vi "GCSTranslator DLL Functions.vi"(0 "System no.":i32=1 min=1 step=1, 1 "Function":T1(ring), 3 "DLL Path (Required for Application, \nmust be set once for the application)":path, 4 "String input":string, 5 "error in":errorcluster, 6 "String buffer":string, 7 "Numerical input":i32, 8 "String input 2":string) -> (14 "DLL I32 Return value":i32, 15 "Boolean output":bool, 16 "String output":string, 17 "Numerical output":i32, 19 "error out":errorcluster)   [LabVIEW 2020]
doc: "This VI calls a given function from GCSTranslator.dll. GCSTranslator.dll must be installed. To call a system-specific function, the system-specific GCS DLL must be installed also. \n\nWarning: For XXX_GcsGetANswer , String buffer must be large enough, otherwise the application may crash. Call XXX_GcsGetANswerSize first to determine necessary string length."
uses:
  Global1.vi
  Global DaisyChain.vi
panel:
  # "This vi calls a given function from GCSTranslator.dll. GCSTranslator.dll must be installed. \nThe system specific GCS DLL must be installed also.\nWARNING: For \"XXXX_GcsGetAnswer\" \"String buffer\" must be large enough, otherwise the \napplication may crash. Call \"XXXX_GcsGetAnswerSize\" first to determine necessary string length."
  # "General inputs:"
  # "Function specific inputs:"
  # "Error handling:"
  # "DLL outputs:"
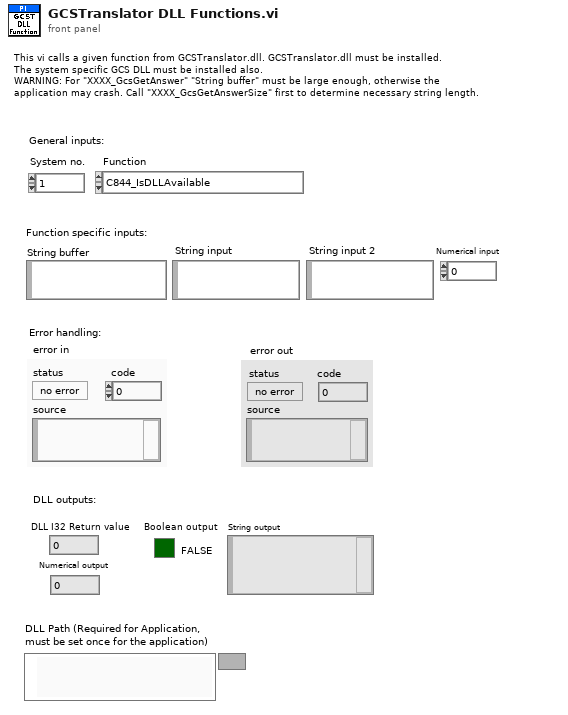
[diagram p1: front panel]
types:
  T1 = enum16{"C844_IsDLLAvailable", "C844_ConnectRS232", "C844_ConnectNIgpib", "C844_IsConnected", "C844_CloseConnection", "C844_GcsCommandset", "C844_GetError", "C844_GcsGetAnswerSize", "C844_GcsGetAnswer", "C843_IsDLLAvailable", "C843_Connect", "C843_IsConnected", "C843_CloseConnection", "C843_GcsCommandset", "C843_GetError", "C843_GcsGetAnswerSize", "C843_GcsGetAnswer", "E710_IsDLLAvailable", "E710_ConnectRS232", "E710_ConnectNIgpib", "E710_IsConnected", "E710_CloseConnection", "E710_GcsCommandset", "E710_GetError", "E710_GcsGetAnswerSize", "E710_GcsGetAnswer", "C843_PM_IsDLLAvailable", "C843_PM_Connect", "C843_PM_IsConnected", "C843_PM_CloseConnection", "C843_PM_GcsCommandset", "C843_PM_GetError", "C843_PM_GcsGetAnswerSize", "C843_PM_GcsGetAnswer", "C843_PM_GetCurrentBoardID", "C843_GetCurrentBoardID", "C865_IsDLLAvailable", "C865_ConnectRS232", "C865_IsConnected", "C865_CloseConnection", "C865_GcsCommandset", "C865_GetError", "C865_GcsGetAnswerSize", "C865_GcsGetAnswer", "C865_GetCurrentInterfaceID", "E761_ConnectPciBoard", "DefineSystem", "CloseConnection", "IsConnected", "ConnectRS232", "ConnectNIgpib", "ConnectPciBoard", "ConnectTCPIP", "GetError", "GcsCommandset", "GCSGetAnswerSize", "GcsGetAnswer", "CloseDaisyChain", "OpenRS232DaisyChain", "ConnectDaisyChainDevice", "ConnectUSB", "ListUSB", "OpenUSBDaisyChain", "OpenTCPIPDaisyChain"}
  T2 = typedef "Available interfaces.ctl" = u16
  T3 = cluster{"RS232 Portnumber":i32, "Timeout":i32, "RS232 Baud rate":u32, "Interface":T2, "GPIB Bus":i32, "GPIB Address":i32, "GPIB Mode":i32}[]
  T4 = cluster{"RS232 Portnumber":i32, "Timeout":i32, "RS232 Baud rate":u32, "Interface":T2, "GPIB Bus":i32, "GPIB Address":i32, "GPIB Mode":i32}
  T5 = typedef "Available DLLs.ctl" = u16
  T6 = typedef "Available DLL interfaces.ctl" = u16
  T7 = cluster{"DLL for Device":T5, "DLL Interface":T6, "Parameter":string}[]
  T8 = cluster{"DLL for Device":T5, "DLL Interface":T6, "Parameter":string}
  T9 = cluster{"No. of devices":i32, "Port ID":i32, "Devices":string[], "Description":string}[]
  T10 = cluster{"No. of devices":i32, "Port ID":i32, "Devices":string[], "Description":string}
  T11 = cluster{"Host address/name":string, "Port":i32, "Board":i32}[]
  T12 = cluster{"Host address/name":string, "Port":i32, "Board":i32}
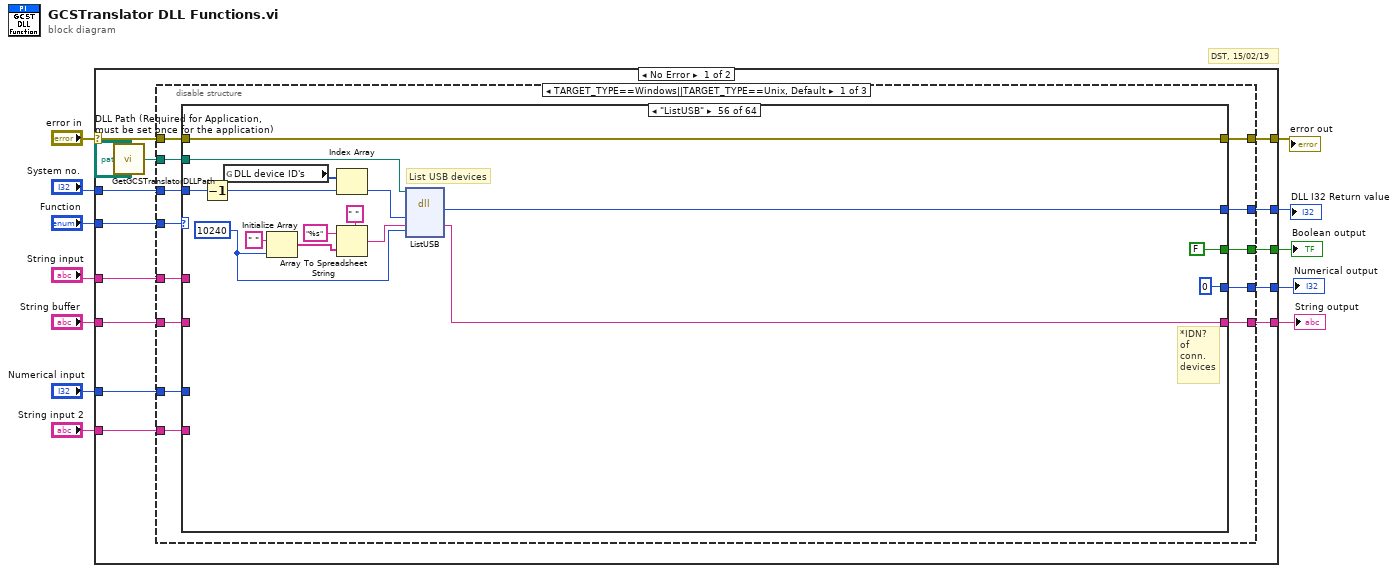
[diagram p0: block diagram]
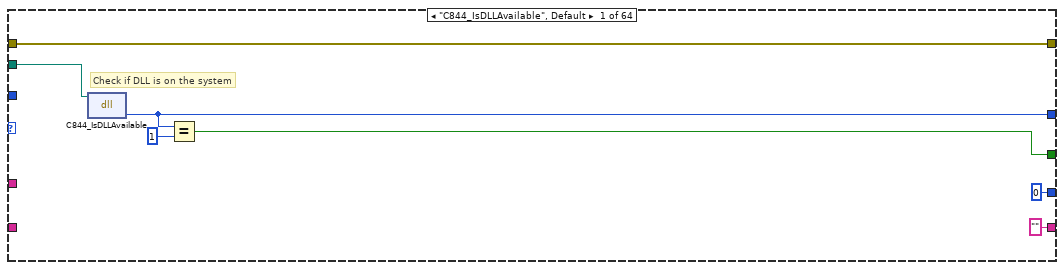
[diagram p2: hidden frame]
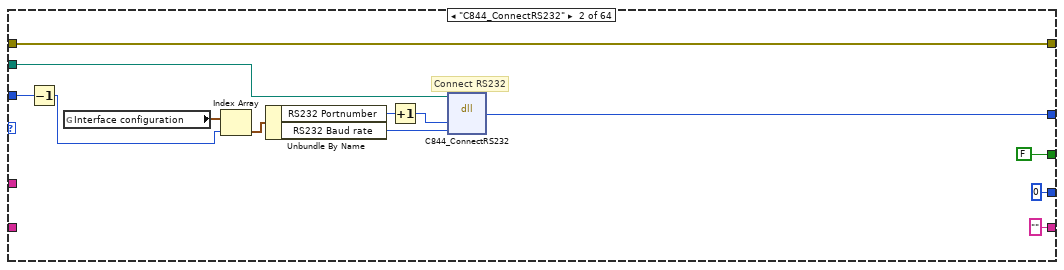
[diagram p3: hidden frame]
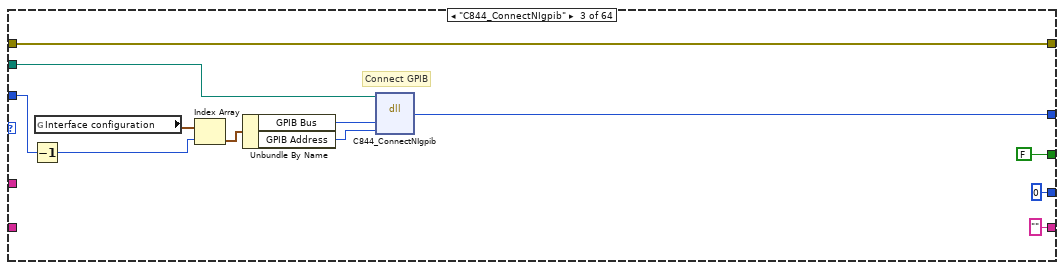
[diagram p4: hidden frame]
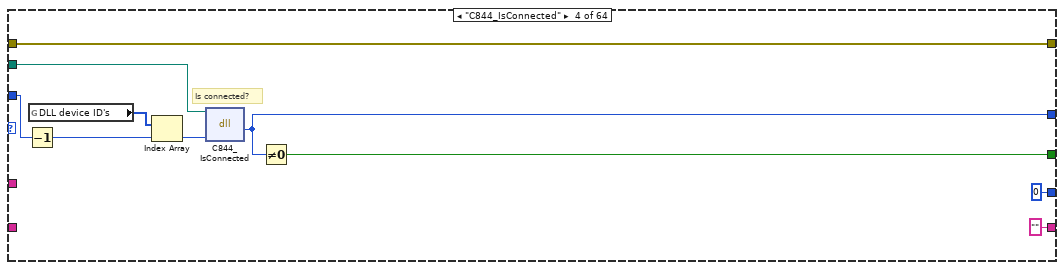
[diagram p5: hidden frame]
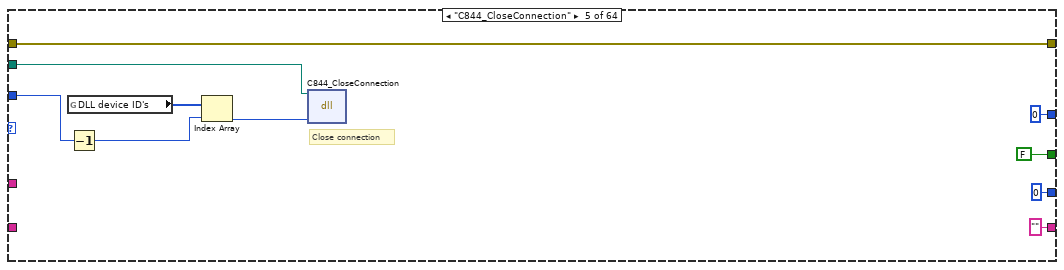
[diagram p6: hidden frame]
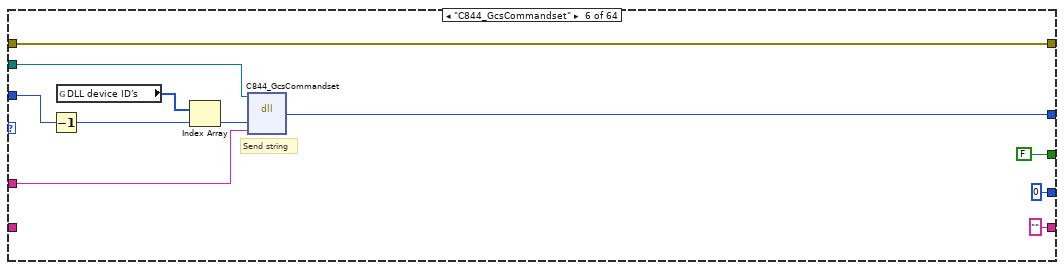
[diagram p7: hidden frame]
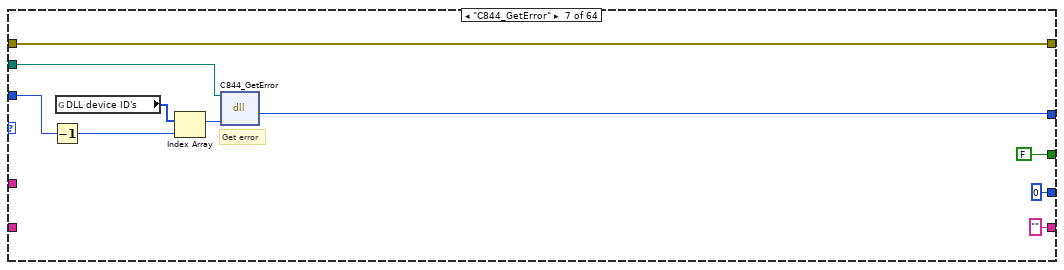
[diagram p8: hidden frame]
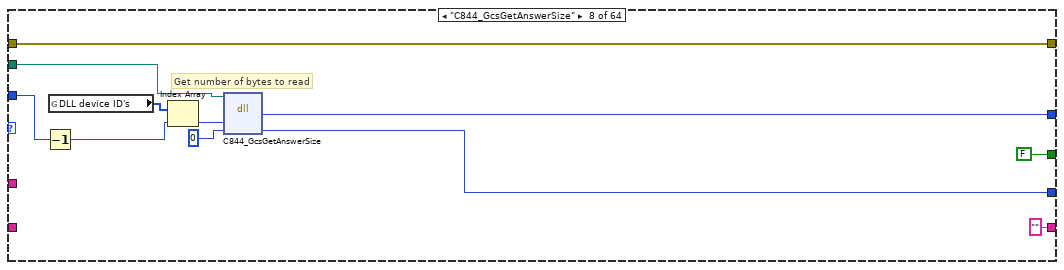
[diagram p9: hidden frame]
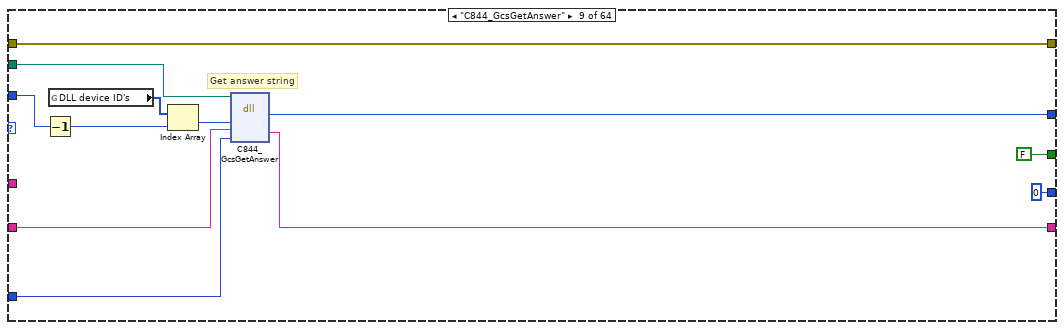
[diagram p10: hidden frame]
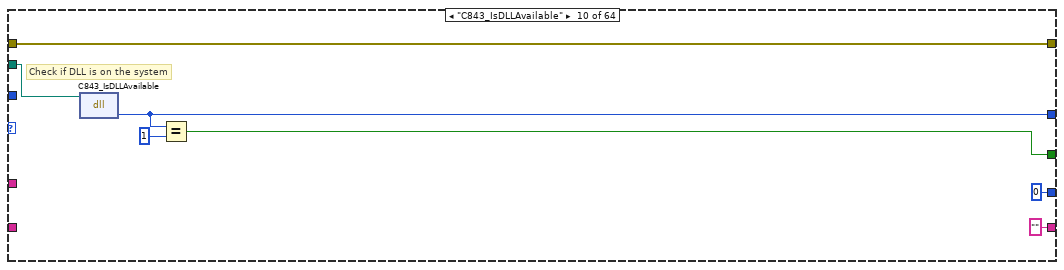
[diagram p11: hidden frame]
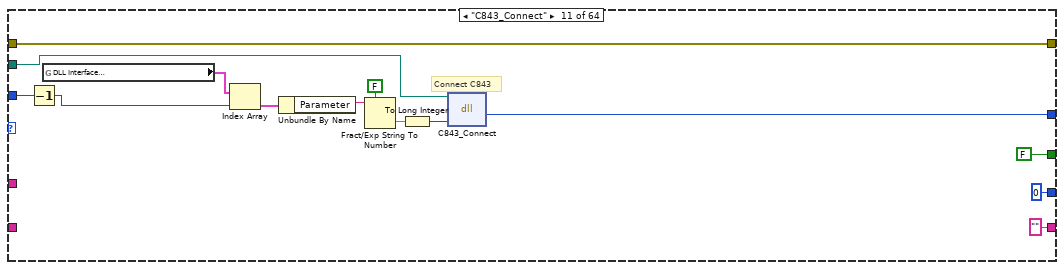
[diagram p12: hidden frame]
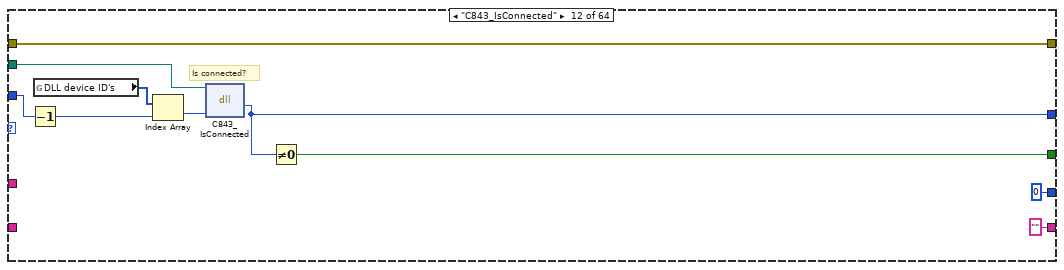
[diagram p13: hidden frame]
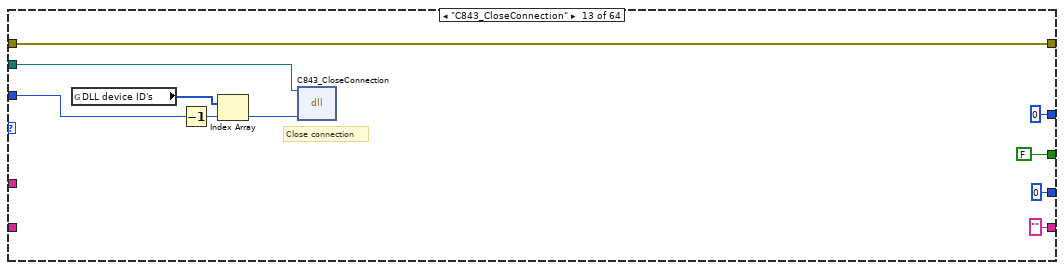
[diagram p14: hidden frame]
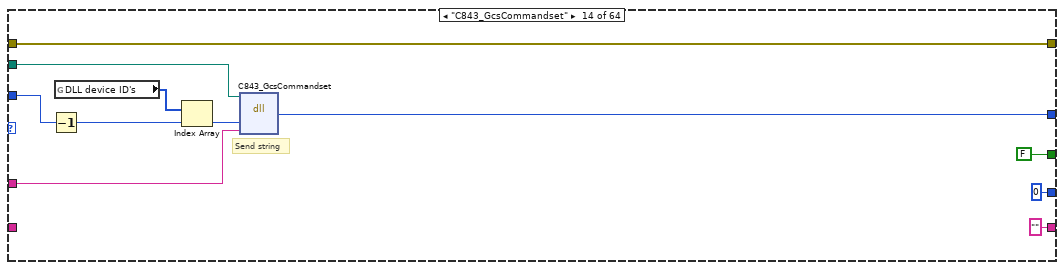
[diagram p15: hidden frame]
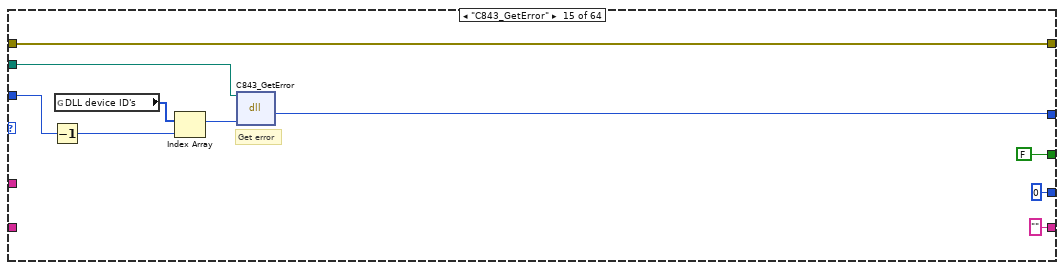
[diagram p16: hidden frame]
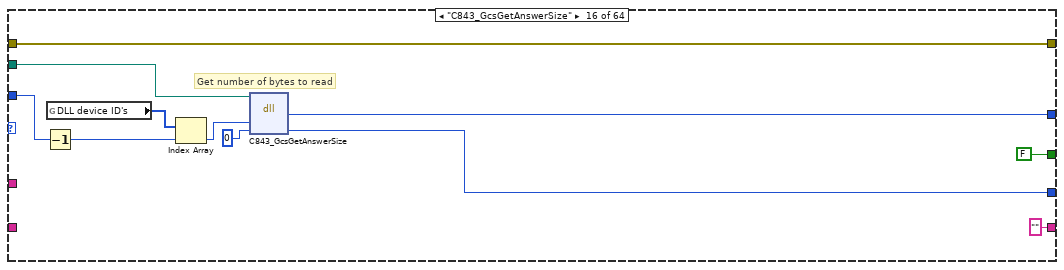
[diagram p17: hidden frame]
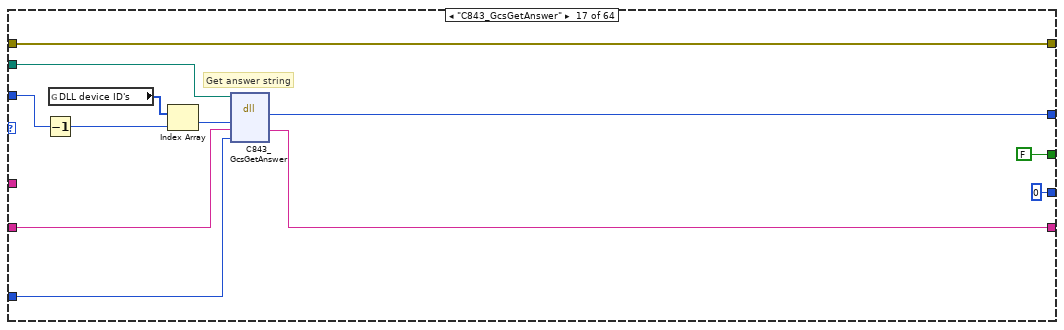
[diagram p18: hidden frame]
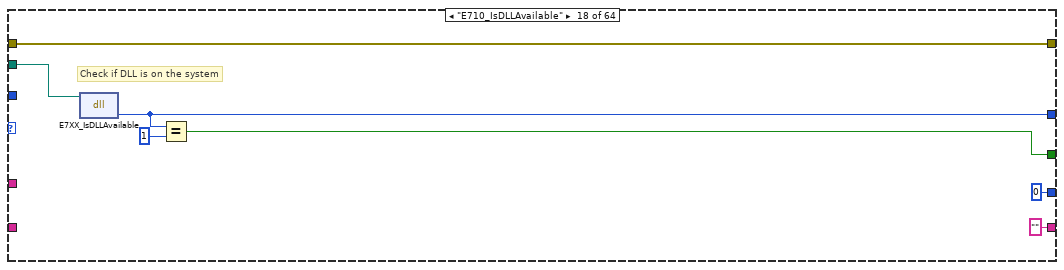
[diagram p19: hidden frame]
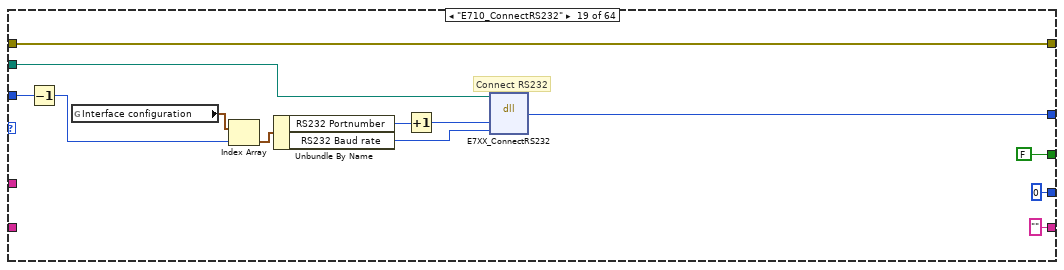
[diagram p20: hidden frame]
diagram:
  # "DST, 15/02/19"
  n1 = case shown="No Error" "error in" {
    selector: "error in" -> [w17 w892]
    tunnel: [w26 w892] -> w12
    tunnel: [w25 0] -> w11
    tunnel: [w24 FALSE] -> w10
    tunnel: "String input" -> [w23 _]
    tunnel: [w22 0 ("iAnswerSize")] -> w8
    tunnel: "String buffer" -> [w21 _]
    tunnel: [w20 "" ("szAnswer")] -> w6
    tunnel: "Numerical input" -> [w19 _]
    tunnel: "String input 2" -> [w18 _]
    tunnel: "System no." -> [w16 _]
    tunnel: "Function" -> [w15 _]
    frame No Error {
      n2 = call "GetGCSTranslatorDLLPath.vi"("DLL Path (Required for Application, \nmust be set once for the application)"="DLL Path (Required for Application, \nmust be set once for the application)") -> ("DLL path"=w14:path)
      n3 = disable-structure shown="TARGET_TYPE==Windows||TARGET_TYPE==Unix, Default" {
        disable-tunnel: w15 -> [w39 _ _]
        disable-tunnel: w17 -> [w38 w890 w891]
        disable-tunnel: [w37 w890 w891] -> w26
        disable-tunnel: [w36 _ _] -> w25
        disable-tunnel: w16 -> [w35 _ _]
        disable-tunnel: [w34 _ _] -> w24
        disable-tunnel: w23 -> [w33 _ _]
        disable-tunnel: [w32 _ _] -> w22
        disable-tunnel: w21 -> [w31 _ _]
        disable-tunnel: [w30 _ _] -> w20
        disable-tunnel: w19 -> [w29 _ _]
        disable-tunnel: w18 -> [w28 _ _]
        disable-tunnel: w14 -> [w27 _ _]
        frame condition #0 (active) {
          n4 = case shown="\"ListUSB\"" w39 {
            tunnel: w35 -> [_ w53 w66 w76 w86 w97 w107 w117 w130 _ w153 w161 w171 w182 w192 w202 w215 _ w234 w247 w257 w267 w278 w288 w298 w311 _ w335 w342 w352 w363 w373 w383 w396 w412 w426 _ w444 w454 w464 w475 w485 w495 w508 w524 _ w540 w548 w583 w600 w622 w651 w701 w734 w763 w779 w791 w807 w821 w835 w846 w861 w871 w884]
            tunnel: w38 -> [w46 w51 w64 w79 w91 w102 w112 w123 w135 w142 w151 w164 w176 w187 w197 w208 w220 w227 w232 w245 w260 w272 w283 w293 w304 w316 w323 w333 w345 w357 w368 w378 w389 w401 w410 w424 w436 w442 w457 w469 w480 w490 w501 w513 w522 w532 w545 w561 w586 w598 w608 w642 w700 w733 w762 w778 w789 w805 w819 w834 w841 w866 w877 w889]
            tunnel: [w46 w51 w64 w79 w91 w102 w112 w123 w135 w142 w151 w164 w176 w187 w197 w208 w220 w227 w232 w245 w260 w272 w283 w293 w304 w316 w323 w333 w345 w357 w368 w378 w389 w401 w410 w424 w436 w442 w457 w469 w480 w490 w501 w513 w522 w532 w545 w561 w586 w598 w607 w641 w700 w733 w762 w778 w789 w805 w819 w834 w840 w866 w877 w889] -> w37
            tunnel: [w45 w52 w65 w78 0 w101 w111 w121 w134 w141 w152 w163 0 w186 w196 w206 w219 w226 w233 w246 w259 0 w282 w292 w302 w315 w322 w334 w344 0 w367 w377 w387 w400 w411 w425 w435 w443 w456 0 w479 w489 w499 w512 w523 w533 0 0 w585 w599 w621 w650 w677 w716 w751 w769 w790 w806 w820 w828 w839 w865 w875 w888] -> w36
            tunnel: [w43 FALSE FALSE w75 FALSE FALSE FALSE FALSE FALSE w139 FALSE w160 FALSE FALSE FALSE FALSE FALSE w224 FALSE FALSE w256 FALSE FALSE FALSE FALSE FALSE w320 FALSE w341 FALSE FALSE FALSE FALSE FALSE FALSE FALSE w433 FALSE w453 FALSE FALSE FALSE FALSE FALSE FALSE FALSE FALSE FALSE w582 FALSE FALSE FALSE FALSE FALSE FALSE FALSE FALSE FALSE FALSE FALSE FALSE FALSE FALSE FALSE] -> w34
            tunnel: w33 -> [_ _ _ _ _ w95 _ _ _ _ _ _ _ w180 _ _ _ _ _ _ _ _ w276 _ _ _ _ _ _ _ w361 _ _ _ _ _ _ _ _ _ w473 _ _ _ _ w535 _ _ _ _ _ _ _ _ _ _ _ _ _ _ _ w859 _ _]
            tunnel: [0 ("iAnswerSize") 0 ("iAnswerSize") 0 ("iAnswerSize") 0 ("iAnswerSize") 0 ("iAnswerSize") 0 ("iAnswerSize") 0 ("iAnswerSize") w115 0 ("iAnswerSize") 0 ("iAnswerSize") 0 ("iAnswerSize") 0 ("iAnswerSize") 0 ("iAnswerSize") 0 ("iAnswerSize") 0 ("iAnswerSize") w200 0 ("iAnswerSize") 0 ("iAnswerSize") 0 ("iAnswerSize") 0 ("iAnswerSize") 0 ("iAnswerSize") 0 ("iAnswerSize") 0 ("iAnswerSize") 0 ("iAnswerSize") w296 0 ("iAnswerSize") 0 ("iAnswerSize") 0 ("iAnswerSize") 0 ("iAnswerSize") 0 ("iAnswerSize") 0 ("iAnswerSize") 0 ("iAnswerSize") w381 0 ("iAnswerSize") 0 ("iAnswerSize") 0 ("iAnswerSize") 0 ("iAnswerSize") 0 ("iAnswerSize") 0 ("iAnswerSize") 0 ("iAnswerSize") 0 ("iAnswerSize") 0 ("iAnswerSize") w493 0 ("iAnswerSize") 0 ("iAnswerSize") 0 ("iAnswerSize") 0 ("iAnswerSize") 0 ("iAnswerSize") 0 ("iAnswerSize") 0 ("iAnswerSize") 0 ("iAnswerSize") 0 ("iAnswerSize") w676 w715 w748 0 ("iAnswerSize") 0 ("iAnswerSize") 0 ("iAnswerSize") 0 ("iAnswerSize") 0 ("iAnswerSize") 0 ("iAnswerSize") 0 ("iAnswerSize") w869 0 ("iAnswerSize")] -> w32
            tunnel: w31 -> [_ _ _ _ _ _ _ _ w128 _ _ _ _ _ _ _ w213 _ _ _ _ _ _ _ _ w309 _ _ _ _ _ _ _ w394 _ _ _ _ _ _ _ _ _ w506 _ _ _ _ _ _ _ _ _ _ _ _ _ _ _ _ _ _ _ w882]
            tunnel: ["" ("szAnswer") "" ("szAnswer") "" ("szAnswer") "" ("szAnswer") "" ("szAnswer") "" ("szAnswer") "" ("szAnswer") "" ("szAnswer") w127 "" ("szAnswer") "" ("szAnswer") "" ("szAnswer") "" ("szAnswer") "" ("szAnswer") "" ("szAnswer") "" ("szAnswer") w212 "" ("szAnswer") "" ("szAnswer") "" ("szAnswer") "" ("szAnswer") "" ("szAnswer") "" ("szAnswer") "" ("szAnswer") "" ("szAnswer") w308 "" ("szAnswer") "" ("szAnswer") "" ("szAnswer") "" ("szAnswer") "" ("szAnswer") "" ("szAnswer") "" ("szAnswer") w393 "" ("szAnswer") "" ("szAnswer") "" ("szAnswer") "" ("szAnswer") "" ("szAnswer") "" ("szAnswer") "" ("szAnswer") "" ("szAnswer") "" ("szAnswer") w505 "" ("szAnswer") "" ("szAnswer") "" ("szAnswer") "" ("szAnswer") "" ("szAnswer") "" ("szAnswer") "" ("szAnswer") "" ("szAnswer") w675 w714 w746 w767 "" ("szAnswer") "" ("szAnswer") "" ("szAnswer") "" ("szAnswer") "" ("szAnswer") "" ("szAnswer") "" ("szAnswer") w881] -> w30
            tunnel: w29 -> [_ _ _ _ _ _ _ _ w125 _ _ _ _ _ _ _ w210 _ _ _ _ _ _ _ _ w306 _ _ _ _ _ _ _ w391 _ _ _ _ _ _ _ _ _ w503 _ _ _ _ _ _ _ _ _ _ _ _ _ _ _ _ _ _ _ w879]
            tunnel: w28 -> [_ _ _ _ _ _ _ _ _ _ _ _ _ _ _ _ _ _ _ _ _ _ _ _ _ _ _ _ _ _ _ _ _ _ _ _ _ _ _ _ _ _ _ _ _ w534 _ _ _ _ _ _ _ _ _ _ _ _ _ _ _ _ _ _]
            tunnel: w27 -> [w40 w47 w60 w72 w82 w92 w103 w113 w124 w136 w143 w157 w167 w177 w188 w198 w209 w221 w228 w241 w253 w263 w273 w284 w294 w305 w317 w324 w338 w348 w358 w369 w379 w390 w402 w416 w430 w437 w450 w460 w470 w481 w491 w502 w514 w528 w536 w546 w579 w589 w604 w631 w666 w705 w737 w764 w780 w794 w810 w824 w838 w856 w867 w878]
            frame "C844_IsDLLAvailable", Default {
              # "Check if DLL is on the system"
              n5 = dll-call lib="T:/Entwicklung/HostSoftware/LabVIEW/GCSDrivers/source/GCS2LabVIEW/Low Level/GCSTranslator.dll" fn="C844_IsDLLAvailable"(path in=w40) -> ("return type"=w45:i32)  [unwired: 2 in, 2 out]
              n6 = Equal?(x=w45, y=1) -> (x = y?=w43:bool)
            }
            frame "C844_ConnectRS232" {
              # "Connect RS232"
              n7 = Decrement(x=w53) -> (x-1=w55:i32)
              n8 = global read "Global1.vi" "Interface configuration"() -> (w56:T3)
              n9 = Index Array(array=w56, index=w55) -> (element=w54:T4)
              n10 = Unbundle By Name(w54) -> ("RS232 Portnumber"=w57:i32, "RS232 Baud rate"=w59:u32)
              n11 = Increment(x=w57) -> (x+1=w58:i32)
              n12 = dll-call lib="T:/Entwicklung/HostSoftware/LabVIEW/GCSDrivers/source/GCS2LabVIEW/Low Level/GCSTranslator.dll" fn="C844_ConnectRS232"(path in=w47, "nPortNr"=w58, "nBaudRate"=w59) -> ("return type"=w52:i32)  [unwired: 4 in, 2 out]
            }
            frame "C844_ConnectNIgpib" {
              # "Connect GPIB"
              n13 = Decrement(x=w66) -> (x-1=w68:i32)
              n14 = global read "Global1.vi" "Interface configuration"() -> (w69:T3)
              n15 = Index Array(array=w69, index=w68) -> (element=w67:T4)
              n16 = Unbundle By Name(w67) -> ("GPIB Bus"=w71:i32, "GPIB Address"=w70:i32)
              n17 = dll-call lib="T:/Entwicklung/HostSoftware/LabVIEW/GCSDrivers/source/GCS2LabVIEW/Low Level/GCSTranslator.dll" fn="C844_ConnectNIgpib"(path in=w60, "nBoard"=w71, "nDevAddr"=w70) -> ("return type"=w65:i32)  [unwired: 4 in, 2 out]
            }
            frame "C844_IsConnected" {
              # "Is connected?"
              n18 = Decrement(x=w76) -> (x-1=w80:i32)
              n19 = global read "Global1.vi" "DLL device ID's"() -> (w77:i32[])
              n20 = Index Array(array=w77, index=w80) -> (element=w81:i32)
              n21 = dll-call lib="T:/Entwicklung/HostSoftware/LabVIEW/GCSDrivers/source/GCS2LabVIEW/Low Level/GCSTranslator.dll" fn="C844_IsConnected"(path in=w72, "ID"=w81) -> ("return type"=w78:i32)  [unwired: 3 in, 2 out]
              n22 = Not Equal To 0?(x=w78) -> (x != 0?=w75:bool)
            }
            frame "C844_CloseConnection" {
              # "Close connection"
              n23 = global read "Global1.vi" "DLL device ID's"() -> (w88:i32[])
              n24 = Decrement(x=w86) -> (x-1=w89:i32)
              n25 = Index Array(array=w88, index=w89) -> (element=w87:i32)
              n26 = dll-call lib="T:/Entwicklung/HostSoftware/LabVIEW/GCSDrivers/source/GCS2LabVIEW/Low Level/GCSTranslator.dll" fn="C844_CloseConnection"(path in=w82, "ID"=w87) -> ()  [unwired: 3 in, 3 out]
            }
            frame "C844_GcsCommandset" {
              # "Send string"
              n27 = Decrement(x=w97) -> (x-1=w100:i32)
              n28 = global read "Global1.vi" "DLL device ID's"() -> (w99:i32[])
              n29 = Index Array(array=w99, index=w100) -> (element=w98:i32)
              n30 = dll-call lib="T:/Entwicklung/HostSoftware/LabVIEW/GCSDrivers/source/GCS2LabVIEW/Low Level/GCSTranslator.dll" fn="C844_GcsCommandset"(path in=w92, "ID"=w98, "szCommand"=w95) -> ("return type"=w101:i32)  [unwired: 4 in, 2 out]
            }
            frame "C844_GetError" {
              # "Get error"
              n31 = Decrement(x=w107) -> (x-1=w110:i32)
              n32 = global read "Global1.vi" "DLL device ID's"() -> (w109:i32[])
              n33 = Index Array(array=w109, index=w110) -> (element=w108:i32)
              n34 = dll-call lib="T:/Entwicklung/HostSoftware/LabVIEW/GCSDrivers/source/GCS2LabVIEW/Low Level/GCSTranslator.dll" fn="C844_GetError"(path in=w103, "ID"=w108) -> ("return type"=w111:i32)  [unwired: 3 in, 2 out]
            }
            frame "C844_GcsGetAnswerSize" {
              # "Get number of bytes to read"
              n35 = Decrement(x=w117) -> (x-1=w120:i32)
              n36 = global read "Global1.vi" "DLL device ID's"() -> (w119:i32[])
              n37 = Index Array(array=w119, index=w120) -> (element=w118:i32)
              n38 = dll-call lib="T:/Entwicklung/HostSoftware/LabVIEW/GCSDrivers/source/GCS2LabVIEW/Low Level/GCSTranslator.dll" fn="C844_GcsGetAnswerSize"(path in=w113, "ID"=w118, "iAnswerSize"=0) -> ("return type"=w121:i32, "iAnswerSize"=w115:i32)  [unwired: 3 in, 2 out]
            }
            frame "C844_GcsGetAnswer" {
              # "Get answer string"
              n39 = Decrement(x=w130) -> (x-1=w133:i32)
              n40 = global read "Global1.vi" "DLL device ID's"() -> (w132:i32[])
              n41 = Index Array(array=w132, index=w133) -> (element=w131:i32)
              n42 = dll-call lib="T:/Entwicklung/HostSoftware/LabVIEW/GCSDrivers/source/GCS2LabVIEW/Low Level/GCSTranslator.dll" fn="C844_GcsGetAnswer"(path in=w124, "ID"=w131, "szAnswer"=w128, "iAnswerSize"=w125) -> ("return type"=w134:i32, "szAnswer"=w127:string)  [unwired: 4 in, 2 out]
            }
            frame "C843_IsDLLAvailable" {
              # "Check if DLL is on the system"
              n43 = dll-call lib="T:/Entwicklung/HostSoftware/LabVIEW/GCSDrivers/source/GCS2LabVIEW/Low Level/GCSTranslator.dll" fn="C843_IsDLLAvailable"(path in=w136) -> ("return type"=w141:i32)  [unwired: 2 in, 2 out]
              n44 = Equal?(x=w141, y=1) -> (x = y?=w139:bool)
            }
            frame "C843_Connect" {
              # "Connect C843"
              n45 = Decrement(x=w153) -> (x-1=w155:i32)
              n46 = global read "Global1.vi" "DLL Interface\nConfiguration"() -> (w156:T7)
              n47 = Index Array(array=w156, index=w155) -> (element=w154:T8)
              n48 = Unbundle By Name(w154) -> ("Parameter"=w147:string)
              n49 = Fract/Exp String To Number(use system decimal point (T)=FALSE, string=w147) -> (number=w148:dbl)  [unwired: 3 out]
              n50 = To Long Integer(number=w148) -> (32bit integer=w146:i32)
              n51 = dll-call lib="T:/Entwicklung/HostSoftware/LabVIEW/GCSDrivers/source/GCS2LabVIEW/Low Level/GCSTranslator.dll" fn="C843_Connect"(path in=w143, "iBoardNumber"=w146) -> ("return type"=w152:i32)  [unwired: 3 in, 2 out]
            }
            frame "C843_IsConnected" {
              # "Is connected?"
              n52 = Decrement(x=w161) -> (x-1=w165:i32)
              n53 = global read "Global1.vi" "DLL device ID's"() -> (w162:i32[])
              n54 = Index Array(array=w162, index=w165) -> (element=w166:i32)
              n55 = dll-call lib="T:/Entwicklung/HostSoftware/LabVIEW/GCSDrivers/source/GCS2LabVIEW/Low Level/GCSTranslator.dll" fn="C843_IsConnected"(path in=w157, "ID"=w166) -> ("return type"=w163:i32)  [unwired: 3 in, 2 out]
              n56 = Not Equal To 0?(x=w163) -> (x != 0?=w160:bool)
            }
            frame "C843_CloseConnection" {
              # "Close connection"
              n57 = global read "Global1.vi" "DLL device ID's"() -> (w173:i32[])
              n58 = Decrement(x=w171) -> (x-1=w174:i32)
              n59 = Index Array(array=w173, index=w174) -> (element=w172:i32)
              n60 = dll-call lib="T:/Entwicklung/HostSoftware/LabVIEW/GCSDrivers/source/GCS2LabVIEW/Low Level/GCSTranslator.dll" fn="C843_CloseConnection"(path in=w167, "ID"=w172) -> ()  [unwired: 3 in, 3 out]
            }
            frame "C843_GcsCommandset" {
              # "Send string"
              n61 = Decrement(x=w182) -> (x-1=w185:i32)
              n62 = global read "Global1.vi" "DLL device ID's"() -> (w184:i32[])
              n63 = Index Array(array=w184, index=w185) -> (element=w183:i32)
              n64 = dll-call lib="T:/Entwicklung/HostSoftware/LabVIEW/GCSDrivers/source/GCS2LabVIEW/Low Level/GCSTranslator.dll" fn="C843_GcsCommandset"(path in=w177, "ID"=w183, "szCommand"=w180) -> ("return type"=w186:i32)  [unwired: 4 in, 2 out]
            }
            frame "C843_GetError" {
              # "Get error"
              n65 = Decrement(x=w192) -> (x-1=w195:i32)
              n66 = global read "Global1.vi" "DLL device ID's"() -> (w194:i32[])
              n67 = Index Array(array=w194, index=w195) -> (element=w193:i32)
              n68 = dll-call lib="T:/Entwicklung/HostSoftware/LabVIEW/GCSDrivers/source/GCS2LabVIEW/Low Level/GCSTranslator.dll" fn="C843_GetError"(path in=w188, "ID"=w193) -> ("return type"=w196:i32)  [unwired: 3 in, 2 out]
            }
            frame "C843_GcsGetAnswerSize" {
              # "Get number of bytes to read"
              n69 = Decrement(x=w202) -> (x-1=w205:i32)
              n70 = global read "Global1.vi" "DLL device ID's"() -> (w204:i32[])
              n71 = Index Array(array=w204, index=w205) -> (element=w203:i32)
              n72 = dll-call lib="T:/Entwicklung/HostSoftware/LabVIEW/GCSDrivers/source/GCS2LabVIEW/Low Level/GCSTranslator.dll" fn="C843_GcsGetAnswerSize"(path in=w198, "ID"=w203, "iAnswerSize"=0) -> ("return type"=w206:i32, "iAnswerSize"=w200:i32)  [unwired: 3 in, 2 out]
            }
            frame "C843_GcsGetAnswer" {
              # "Get answer string"
              n73 = Decrement(x=w215) -> (x-1=w218:i32)
              n74 = global read "Global1.vi" "DLL device ID's"() -> (w217:i32[])
              n75 = Index Array(array=w217, index=w218) -> (element=w216:i32)
              n76 = dll-call lib="T:/Entwicklung/HostSoftware/LabVIEW/GCSDrivers/source/GCS2LabVIEW/Low Level/GCSTranslator.dll" fn="C843_GcsGetAnswer"(path in=w209, "ID"=w216, "szAnswer"=w213, "iAnswerSize"=w210) -> ("return type"=w219:i32, "szAnswer"=w212:string)  [unwired: 4 in, 2 out]
            }
            frame "E710_IsDLLAvailable" {
              # "Check if DLL is on the system"
              n77 = dll-call lib="T:/Entwicklung/HostSoftware/LabVIEW/GCSDrivers/source/GCS2LabVIEW/Low Level/GCSTranslator.dll" fn="E7XX_IsDLLAvailable"(path in=w221) -> ("return type"=w226:i32)  [unwired: 2 in, 2 out]
              n78 = Equal?(x=w226, y=1) -> (x = y?=w224:bool)
            }
            frame "E710_ConnectRS232" {
              # "Connect RS232"
              n79 = Decrement(x=w234) -> (x-1=w236:i32)
              n80 = global read "Global1.vi" "Interface configuration"() -> (w237:T3)
              n81 = Index Array(array=w237, index=w236) -> (element=w235:T4)
              n82 = Unbundle By Name(w235) -> ("RS232 Portnumber"=w238:i32, "RS232 Baud rate"=w240:u32)
              n83 = Increment(x=w238) -> (x+1=w239:i32)
              n84 = dll-call lib="T:/Entwicklung/HostSoftware/LabVIEW/GCSDrivers/source/GCS2LabVIEW/Low Level/GCSTranslator.dll" fn="E7XX_ConnectRS232"(path in=w228, "nPortNr"=w239, "nBaudRate"=w240) -> ("return type"=w233:i32)  [unwired: 4 in, 2 out]
            }
            frame "E710_ConnectNIgpib" {
              # "Connect GPIB"
              n85 = Decrement(x=w247) -> (x-1=w249:i32)
              n86 = global read "Global1.vi" "Interface configuration"() -> (w250:T3)
              n87 = Index Array(array=w250, index=w249) -> (element=w248:T4)
              n88 = Unbundle By Name(w248) -> ("GPIB Bus"=w252:i32, "GPIB Address"=w251:i32)
              n89 = dll-call lib="T:/Entwicklung/HostSoftware/LabVIEW/GCSDrivers/source/GCS2LabVIEW/Low Level/GCSTranslator.dll" fn="E7XX_ConnectNIgpib"(path in=w241, "nBoard"=w252, "nDevAddr"=w251) -> ("return type"=w246:i32)  [unwired: 4 in, 2 out]
            }
            frame "E710_IsConnected" {
              # "Is connected?"
              n90 = global read "Global1.vi" "DLL device ID's"() -> (w258:i32[])
              n91 = Decrement(x=w257) -> (x-1=w261:i32)
              n92 = Index Array(array=w258, index=w261) -> (element=w262:i32)
              n93 = dll-call lib="T:/Entwicklung/HostSoftware/LabVIEW/GCSDrivers/source/GCS2LabVIEW/Low Level/GCSTranslator.dll" fn="E7XX_IsConnected"(path in=w253, "ID"=w262) -> ("return type"=w259:i32)  [unwired: 3 in, 2 out]
              n94 = Not Equal To 0?(x=w259) -> (x != 0?=w256:bool)
            }
            frame "E710_CloseConnection" {
              # "Close connection"
              n95 = global read "Global1.vi" "DLL device ID's"() -> (w269:i32[])
              n96 = Decrement(x=w267) -> (x-1=w270:i32)
              n97 = Index Array(array=w269, index=w270) -> (element=w268:i32)
              n98 = dll-call lib="T:/Entwicklung/HostSoftware/LabVIEW/GCSDrivers/source/GCS2LabVIEW/Low Level/GCSTranslator.dll" fn="E7XX_CloseConnection"(path in=w263, "ID"=w268) -> ()  [unwired: 3 in, 3 out]
            }
            frame "E710_GcsCommandset" {
              # "Send string"
              n99 = global read "Global1.vi" "DLL device ID's"() -> (w280:i32[])
              n100 = Decrement(x=w278) -> (x-1=w281:i32)
              n101 = Index Array(array=w280, index=w281) -> (element=w279:i32)
              n102 = dll-call lib="T:/Entwicklung/HostSoftware/LabVIEW/GCSDrivers/source/GCS2LabVIEW/Low Level/GCSTranslator.dll" fn="E7XX_GcsCommandset"(path in=w273, "ID"=w279, "szCommand"=w276) -> ("return type"=w282:i32)  [unwired: 4 in, 2 out]
            }
            frame "E710_GetError" {
              # "Get error"
              n103 = Decrement(x=w288) -> (x-1=w291:i32)
              n104 = global read "Global1.vi" "DLL device ID's"() -> (w290:i32[])
              n105 = Index Array(array=w290, index=w291) -> (element=w289:i32)
              n106 = dll-call lib="T:/Entwicklung/HostSoftware/LabVIEW/GCSDrivers/source/GCS2LabVIEW/Low Level/GCSTranslator.dll" fn="E7XX_GetError"(path in=w284, "ID"=w289) -> ("return type"=w292:i32)  [unwired: 3 in, 2 out]
            }
            frame "E710_GcsGetAnswerSize" {
              # "Get number of bytes to read"
              n107 = Decrement(x=w298) -> (x-1=w301:i32)
              n108 = global read "Global1.vi" "DLL device ID's"() -> (w300:i32[])
              n109 = Index Array(array=w300, index=w301) -> (element=w299:i32)
              n110 = dll-call lib="T:/Entwicklung/HostSoftware/LabVIEW/GCSDrivers/source/GCS2LabVIEW/Low Level/GCSTranslator.dll" fn="E7XX_GcsGetAnswerSize"(path in=w294, "ID"=w299, "iAnswerSize"=0) -> ("return type"=w302:i32, "iAnswerSize"=w296:i32)  [unwired: 3 in, 2 out]
            }
            frame "E710_GcsGetAnswer" {
              # "Get answer string"
              n111 = Decrement(x=w311) -> (x-1=w314:i32)
              n112 = global read "Global1.vi" "DLL device ID's"() -> (w313:i32[])
              n113 = Index Array(array=w313, index=w314) -> (element=w312:i32)
              n114 = dll-call lib="T:/Entwicklung/HostSoftware/LabVIEW/GCSDrivers/source/GCS2LabVIEW/Low Level/GCSTranslator.dll" fn="E7XX_GcsGetAnswer"(path in=w305, "ID"=w312, "szAnswer"=w309, "iAnswerSize"=w306) -> ("return type"=w315:i32, "szAnswer"=w308:string)  [unwired: 4 in, 2 out]
            }
            frame "C843_PM_IsDLLAvailable" {
              # "Check if DLL is on the system"
              n115 = dll-call lib="T:/Entwicklung/HostSoftware/LabVIEW/GCSDrivers/source/GCS2LabVIEW/Low Level/GCSTranslator.dll" fn="C843_PM_IsDLLAvailable"(path in=w317) -> ("return type"=w322:i32)  [unwired: 2 in, 2 out]
              n116 = Equal?(x=w322, y=1) -> (x = y?=w320:bool)
            }
            frame "C843_PM_Connect" {
              # "Connect C843_PM"
              n117 = Decrement(x=w335) -> (x-1=w325:i32)
              n118 = global read "Global1.vi" "DLL Interface\nConfiguration"() -> (w337:T7)
              n119 = Index Array(array=w337, index=w325) -> (element=w336:T8)
              n120 = Unbundle By Name(w336) -> ("Parameter"=w329:string)
              n121 = Fract/Exp String To Number(use system decimal point (T)=FALSE, string=w329) -> (number=w330:dbl)  [unwired: 3 out]
              n122 = To Long Integer(number=w330) -> (32bit integer=w328:i32)
              n123 = dll-call lib="T:/Entwicklung/HostSoftware/LabVIEW/GCSDrivers/source/GCS2LabVIEW/Low Level/GCSTranslator.dll" fn="C843_PM_Connect"(path in=w324, "iBoardNumber"=w328) -> ("return type"=w334:i32)  [unwired: 3 in, 2 out]
            }
            frame "C843_PM_IsConnected" {
              # "Is connected?"
              n124 = Decrement(x=w342) -> (x-1=w346:i32)
              n125 = global read "Global1.vi" "DLL device ID's"() -> (w343:i32[])
              n126 = Index Array(array=w343, index=w346) -> (element=w347:i32)
              n127 = dll-call lib="T:/Entwicklung/HostSoftware/LabVIEW/GCSDrivers/source/GCS2LabVIEW/Low Level/GCSTranslator.dll" fn="C843_PM_IsConnected"(path in=w338, "ID"=w347) -> ("return type"=w344:i32)  [unwired: 3 in, 2 out]
              n128 = Not Equal To 0?(x=w344) -> (x != 0?=w341:bool)
            }
            frame "C843_PM_CloseConnection" {
              # "Close connection"
              n129 = Decrement(x=w352) -> (x-1=w355:i32)
              n130 = global read "Global1.vi" "DLL device ID's"() -> (w354:i32[])
              n131 = Index Array(array=w354, index=w355) -> (element=w353:i32)
              n132 = dll-call lib="T:/Entwicklung/HostSoftware/LabVIEW/GCSDrivers/source/GCS2LabVIEW/Low Level/GCSTranslator.dll" fn="C843_PM_CloseConnection"(path in=w348, "ID"=w353) -> ()  [unwired: 3 in, 3 out]
            }
            frame "C843_PM_GcsCommandset" {
              # "Send string"
              n133 = Decrement(x=w363) -> (x-1=w366:i32)
              n134 = global read "Global1.vi" "DLL device ID's"() -> (w365:i32[])
              n135 = Index Array(array=w365, index=w366) -> (element=w364:i32)
              n136 = dll-call lib="T:/Entwicklung/HostSoftware/LabVIEW/GCSDrivers/source/GCS2LabVIEW/Low Level/GCSTranslator.dll" fn="C843_PM_GcsCommandset"(path in=w358, "ID"=w364, "szCommand"=w361) -> ("return type"=w367:i32)  [unwired: 4 in, 2 out]
            }
            frame "C843_PM_GetError" {
              # "Get error"
              n137 = Decrement(x=w373) -> (x-1=w376:i32)
              n138 = global read "Global1.vi" "DLL device ID's"() -> (w375:i32[])
              n139 = Index Array(array=w375, index=w376) -> (element=w374:i32)
              n140 = dll-call lib="T:/Entwicklung/HostSoftware/LabVIEW/GCSDrivers/source/GCS2LabVIEW/Low Level/GCSTranslator.dll" fn="C843_PM_GetError"(path in=w369, "ID"=w374) -> ("return type"=w377:i32)  [unwired: 3 in, 2 out]
            }
            frame "C843_PM_GcsGetAnswerSize" {
              # "Get number of bytes to read"
              n141 = Decrement(x=w383) -> (x-1=w386:i32)
              n142 = global read "Global1.vi" "DLL device ID's"() -> (w385:i32[])
              n143 = Index Array(array=w385, index=w386) -> (element=w384:i32)
              n144 = dll-call lib="T:/Entwicklung/HostSoftware/LabVIEW/GCSDrivers/source/GCS2LabVIEW/Low Level/GCSTranslator.dll" fn="C843_PM_GcsGetAnswerSize"(path in=w379, "ID"=w384, "iAnswerSize"=0) -> ("return type"=w387:i32, "iAnswerSize"=w381:i32)  [unwired: 3 in, 2 out]
            }
            frame "C843_PM_GcsGetAnswer" {
              # "Get answer string"
              n145 = Decrement(x=w396) -> (x-1=w399:i32)
              n146 = global read "Global1.vi" "DLL device ID's"() -> (w398:i32[])
              n147 = Index Array(array=w398, index=w399) -> (element=w397:i32)
              n148 = dll-call lib="T:/Entwicklung/HostSoftware/LabVIEW/GCSDrivers/source/GCS2LabVIEW/Low Level/GCSTranslator.dll" fn="C843_PM_GcsGetAnswer"(path in=w390, "ID"=w397, "szAnswer"=w394, "iAnswerSize"=w391) -> ("return type"=w400:i32, "szAnswer"=w393:string)  [unwired: 4 in, 2 out]
            }
            frame "C843_PM_GetCurrentBoardID" {
              # "Get current ID C843_PM"
              n149 = Decrement(x=w412) -> (x-1=w414:i32)
              n150 = global read "Global1.vi" "DLL Interface\nConfiguration"() -> (w415:T7)
              n151 = Index Array(array=w415, index=w414) -> (element=w413:T8)
              n152 = Unbundle By Name(w413) -> ("Parameter"=w406:string)
              n153 = Fract/Exp String To Number(use system decimal point (T)=FALSE, string=w406) -> (number=w407:dbl)  [unwired: 3 out]
              n154 = To Long Integer(number=w407) -> (32bit integer=w405:i32)
              n155 = dll-call lib="T:/Entwicklung/HostSoftware/LabVIEW/GCSDrivers/source/GCS2LabVIEW/Low Level/GCSTranslator.dll" fn="C843_PM_GetCurrentBoardId"(path in=w402, "iBoardNumber"=w405) -> ("return type"=w411:i32)  [unwired: 3 in, 2 out]
            }
            frame "C843_GetCurrentBoardID" {
              # "Get current ID C843"
              n156 = Decrement(x=w426) -> (x-1=w428:i32)
              n157 = global read "Global1.vi" "DLL Interface\nConfiguration"() -> (w429:T7)
              n158 = Index Array(array=w429, index=w428) -> (element=w427:T8)
              n159 = Unbundle By Name(w427) -> ("Parameter"=w420:string)
              n160 = Fract/Exp String To Number(use system decimal point (T)=FALSE, string=w420) -> (number=w421:dbl)  [unwired: 3 out]
              n161 = To Long Integer(number=w421) -> (32bit integer=w419:i32)
              n162 = dll-call lib="T:/Entwicklung/HostSoftware/LabVIEW/GCSDrivers/source/GCS2LabVIEW/Low Level/GCSTranslator.dll" fn="C843_GetCurrentBoardId"(path in=w416, "iBoardNumber"=w419) -> ("return type"=w425:i32)  [unwired: 3 in, 2 out]
            }
            frame "C865_IsDLLAvailable" {
              # "Check if DLL is on the system"
              n163 = dll-call lib="T:/Entwicklung/HostSoftware/LabVIEW/GCSDrivers/source/GCS2LabVIEW/Low Level/GCSTranslator.dll" fn="C865_IsDLLAvailable"(path in=w430) -> ("return type"=w435:i32)  [unwired: 2 in, 2 out]
              n164 = Equal?(x=w435, y=1) -> (x = y?=w433:bool)
            }
            frame "C865_ConnectRS232" {
              # "Connect RS232"
              n165 = Decrement(x=w444) -> (x-1=w438:i32)
              n166 = global read "Global1.vi" "Interface configuration"() -> (w446:T3)
              n167 = Index Array(array=w446, index=w438) -> (element=w445:T4)
              n168 = Unbundle By Name(w445) -> ("RS232 Portnumber"=w447:i32, "RS232 Baud rate"=w449:u32)
              n169 = Increment(x=w447) -> (x+1=w448:i32)
              n170 = dll-call lib="T:/Entwicklung/HostSoftware/LabVIEW/GCSDrivers/source/GCS2LabVIEW/Low Level/GCSTranslator.dll" fn="C865_ConnectRS232"(path in=w437, "nPortNr"=w448, "nBaudRate"=w449) -> ("return type"=w443:i32)  [unwired: 4 in, 2 out]
            }
            frame "C865_IsConnected" {
              # "Is connected?"
              n171 = global read "Global1.vi" "DLL device ID's"() -> (w455:i32[])
              n172 = Decrement(x=w454) -> (x-1=w458:i32)
              n173 = Index Array(array=w455, index=w458) -> (element=w459:i32)
              n174 = dll-call lib="T:/Entwicklung/HostSoftware/LabVIEW/GCSDrivers/source/GCS2LabVIEW/Low Level/GCSTranslator.dll" fn="C865_IsConnected"(path in=w450, "ID"=w459) -> ("return type"=w456:i32)  [unwired: 3 in, 2 out]
              n175 = Not Equal To 0?(x=w456) -> (x != 0?=w453:bool)
            }
            frame "C865_CloseConnection" {
              # "Close connection"
              n176 = global read "Global1.vi" "DLL device ID's"() -> (w466:i32[])
              n177 = Decrement(x=w464) -> (x-1=w467:i32)
              n178 = Index Array(array=w466, index=w467) -> (element=w465:i32)
              n179 = dll-call lib="T:/Entwicklung/HostSoftware/LabVIEW/GCSDrivers/source/GCS2LabVIEW/Low Level/GCSTranslator.dll" fn="C865_CloseConnection"(path in=w460, "ID"=w465) -> ()  [unwired: 3 in, 3 out]
            }
            frame "C865_GcsCommandset" {
              # "Send string"
              n180 = global read "Global1.vi" "DLL device ID's"() -> (w477:i32[])
              n181 = Decrement(x=w475) -> (x-1=w478:i32)
              n182 = Index Array(array=w477, index=w478) -> (element=w476:i32)
              n183 = dll-call lib="T:/Entwicklung/HostSoftware/LabVIEW/GCSDrivers/source/GCS2LabVIEW/Low Level/GCSTranslator.dll" fn="C865_GcsCommandset"(path in=w470, "ID"=w476, "szCommand"=w473) -> ("return type"=w479:i32)  [unwired: 4 in, 2 out]
            }
            frame "C865_GetError" {
              # "Get error"
              n184 = Decrement(x=w485) -> (x-1=w488:i32)
              n185 = global read "Global1.vi" "DLL device ID's"() -> (w487:i32[])
              n186 = Index Array(array=w487, index=w488) -> (element=w486:i32)
              n187 = dll-call lib="T:/Entwicklung/HostSoftware/LabVIEW/GCSDrivers/source/GCS2LabVIEW/Low Level/GCSTranslator.dll" fn="C865_GetError"(path in=w481, "ID"=w486) -> ("return type"=w489:i32)  [unwired: 3 in, 2 out]
            }
            frame "C865_GcsGetAnswerSize" {
              # "Get number of bytes to read"
              n188 = global read "Global1.vi" "DLL device ID's"() -> (w497:i32[])
              n189 = Decrement(x=w495) -> (x-1=w498:i32)
              n190 = Index Array(array=w497, index=w498) -> (element=w496:i32)
              n191 = dll-call lib="T:/Entwicklung/HostSoftware/LabVIEW/GCSDrivers/source/GCS2LabVIEW/Low Level/GCSTranslator.dll" fn="C865_GcsGetAnswerSize"(path in=w491, "ID"=w496, "iAnswerSize"=0) -> ("return type"=w499:i32, "iAnswerSize"=w493:i32)  [unwired: 3 in, 2 out]
            }
            frame "C865_GcsGetAnswer" {
              # "Get answer string"
              n192 = Decrement(x=w508) -> (x-1=w511:i32)
              n193 = global read "Global1.vi" "DLL device ID's"() -> (w510:i32[])
              n194 = Index Array(array=w510, index=w511) -> (element=w509:i32)
              n195 = dll-call lib="T:/Entwicklung/HostSoftware/LabVIEW/GCSDrivers/source/GCS2LabVIEW/Low Level/GCSTranslator.dll" fn="C865_GcsGetAnswer"(path in=w502, "ID"=w509, "szAnswer"=w506, "iAnswerSize"=w503) -> ("return type"=w512:i32, "szAnswer"=w505:string)  [unwired: 4 in, 2 out]
            }
            frame "C865_GetCurrentInterfaceID" {
              # "Get current ID C865"
              n196 = Decrement(x=w524) -> (x-1=w526:i32)
              n197 = global read "Global1.vi" "DLL Interface\nConfiguration"() -> (w527:T7)
              n198 = Index Array(array=w527, index=w526) -> (element=w525:T8)
              n199 = Unbundle By Name(w525) -> ("Parameter"=w518:string)
              n200 = Fract/Exp String To Number(use system decimal point (T)=FALSE, string=w518) -> (number=w519:dbl)  [unwired: 3 out]
              n201 = To Long Integer(number=w519) -> (32bit integer=w517:i32)
              n202 = dll-call lib="T:/Entwicklung/HostSoftware/LabVIEW/GCSDrivers/source/GCS2LabVIEW/Low Level/GCSTranslator.dll" fn="C865_GetCurrentInterfaceId"(path in=w514, "iBoardNumber"=w517) -> ("return type"=w523:i32)  [unwired: 3 in, 2 out]
            }
            frame "DefineSystem" {
              # "Define which GCS dll to use and for which system"
              n203 = dll-call lib="T:/Entwicklung/HostSoftware/LabVIEW/GCSDrivers/source/GCS2LabVIEW/Low Level/GCSTranslator.dll" fn="DefineSystem"(path in=w528, "szDLLName"=w535, "szCtrlPrefix"=w534) -> ("return type"=w533:i32)  [unwired: 4 in, 2 out]
            }
            frame "CloseConnection" {
              # "Close connection"
              n204 = global read "Global1.vi" "DLL device ID's"() -> (w542:i32[])
              n205 = Decrement(x=w540) -> (x-1=w543:i32)
              n206 = Index Array(array=w542, index=w543) -> (element=w541:i32)
              n207 = dll-call lib="T:/Entwicklung/HostSoftware/LabVIEW/GCSDrivers/source/GCS2LabVIEW/Low Level/GCSTranslator.dll" fn="CloseConnection"(path in=w536, "ID"=w541) -> ()  [unwired: 3 in, 3 out]
            }
            frame "CloseDaisyChain" {
              # "CloseDaisyChain"
              n208 = Decrement(x=w548) -> (x-1=w553:i32)
              n209 = global read "Global1.vi" "DLL device ID's"() -> (w559:i32[])
              n210 = global read "Global DaisyChain.vi" "DaisyChain configuration"() -> (w551:T9)
              n211 = global read "Global1.vi" "Number of\nsystems"() -> (w549:i32)
              n212 = Index Array(array=w559, index=w553) -> (element=w558:i32)
              n213 = Max & Min(x=w548, y=w549) -> (max(x,y)=w547:i32)  [unwired: 1 out]
              n214 = Index Array(array=w551, index=w553) -> (element=w554:T10)
              n215 = Unbundle By Name(w554) -> ("Port ID"=w552:i32)
              n216 = for {
                N: w547 -> [_]
                tunnel: w551 -> [w567]
                shift-right: [w569] -> w550
                shift-left: w551 -> [w568]
                tunnel: w552 -> [w565]
                i -> [w563]
                n217 = Index Array(array=w567, index=w563) -> (element=w562:T10)
                n218 = Unbundle By Name(w562) -> ("Port ID"=w566:i32)
                n219 = Equal?(x=w566, y=w565) -> (x = y?=w564:bool)
                n220 = case shown="True" w564 {
                  tunnel: [w570 w575] -> w569
                  tunnel: w568 -> [w570 w573]
                  tunnel: w563 -> [_ w574]
                  tunnel: w562 -> [_ w572]
                  frame False {
                  }
                  frame True {
                    n221 = Bundle By Name(cluster=w572, "Port ID"=-1, "No. of devices"=0, "Devices"=string[] []) -> (w571:T10)
                    n222 = Replace Array Subset(array=w573, new element=w571, index=w574) -> (w575:T9)
                  }
                }
              }
              n223 = dll-call lib="T:/Entwicklung/HostSoftware/LabVIEW/GCSDrivers/source/GCS2LabVIEW/Low Level/GCSTranslator.dll" fn="CloseDaisyChain"(path in=w546, "ID"=w558, "iPortID"=w552) -> ()  [unwired: 4 in, 3 out]
              n224 = global write "Global DaisyChain.vi" "DaisyChain configuration"(w550) -> ()
            }
            frame "IsConnected" {
              # "Is connected?"
              n225 = global read "Global1.vi" "DLL device ID's"() -> (w584:i32[])
              n226 = Decrement(x=w583) -> (x-1=w587:i32)
              n227 = Index Array(array=w584, index=w587) -> (element=w588:i32)
              n228 = dll-call lib="T:/Entwicklung/HostSoftware/LabVIEW/GCSDrivers/source/GCS2LabVIEW/Low Level/GCSTranslator.dll" fn="IsConnected"(path in=w579, "ID"=w588) -> ("return type"=w585:i32)  [unwired: 3 in, 2 out]
              n229 = Not Equal To 0?(x=w585) -> (x != 0?=w582:bool)
            }
            frame "ConnectRS232" {
              # "Port ID"
              # "Connect RS232"
              n230 = Decrement(x=w600) -> (x-1=w591:i32)
              n231 = global read "Global1.vi" "DLL device ID's"() -> (w592:i32[])
              n232 = global read "Global1.vi" "Interface configuration"() -> (w602:T3)
              n233 = Index Array(array=w592, index=w591) -> (element=w590:i32)
              n234 = Index Array(array=w602, index=w591) -> (element=w601:T4)
              n235 = Unbundle By Name(w601) -> ("RS232 Portnumber"=w603:i32, "RS232 Baud rate"=w594:u32)
              n236 = Increment(x=w603) -> (x+1=w593:i32)
              n237 = dll-call lib="T:/Entwicklung/HostSoftware/LabVIEW/GCSDrivers/source/GCS2LabVIEW/Low Level/GCSTranslator.dll" fn="ConnectRS232"(path in=w589, "ID"=w590, "nPortNr"=w593, "nBaudRate"=w594) -> ("return type"=w599:i32)  [unwired: 5 in, 2 out]
            }
            frame "ConnectDaisyChainDevice" {
              # "Connect DaisyChainDevice"
              n238 = Decrement(x=w622) -> (x-1=w611:i32)
              n239 = global read "Global1.vi" "DLL device ID's"() -> (w617:i32[])
              n240 = global read "Global DaisyChain.vi" "DaisyChain configuration"() -> (w615:T9)
              n241 = Index Array(array=w617, index=w611) -> (element=w616:i32)
              n242 = Index Array(array=w615, index=w611) -> (element=w614:T10)
              n243 = Unbundle By Name(w614) -> ("Port ID"=w610:i32, "Description"=w605:string)
              n244 = Fract/Exp String To Number(use system decimal point (T)=FALSE, string=w605) -> (number=w612:dbl)  [unwired: 3 out]
              n245 = Less Than 0?(x=w610) -> (x < 0?=w606:bool)
              n246 = To Long Integer(number=w612) -> (32bit integer=w609:i32)
              n247 = case shown="False" w606 {
                tunnel: [w628 -1] -> w621
                tunnel: w616 -> [w627 _]
                tunnel: w609 -> [w626 _]
                tunnel: w610 -> [w625 _]
                tunnel: [w624 errorcluster {"status"=TRUE, "code"=100, "source"="Check DeviceID, cable\nconnections and\nbaudrate settings."} ("error in")] -> w607
                tunnel: w608 -> [w624 _]
                tunnel: w604 -> [w623 _]
                frame False {
                  n248 = dll-call lib="T:/Entwicklung/HostSoftware/LabVIEW/GCSDrivers/source/GCS2LabVIEW/Low Level/GCSTranslator.dll" fn="ConnectDaisyChainDevice"(path in=w623, "ID"=w627, "iPortId"=w625, "iDeviceNumber"=w626) -> ("return type"=w628:i32)  [unwired: 5 in, 2 out]
                }
                frame True {
                }
              }
            }
            frame "ConnectUSB" {
              # "ConnectUSB"
              n249 = Decrement(x=w651) -> (x-1=w635:i32)
              n250 = global read "Global1.vi" "DLL device ID's"() -> (w646:i32[])
              n251 = global read "Global1.vi" "DLL Interface\nConfiguration"() -> (w644:T7)
              n252 = global read "Global DaisyChain.vi" "DaisyChain configuration"() -> (w634:T9)
              n253 = Index Array(array=w646, index=w635) -> (element=w645:i32)
              n254 = Index Array(array=w644, index=w635) -> (element=w643:T8)
              n255 = Index Array(array=w634, index=w635) -> (element=w633:T10)
              n256 = Unbundle By Name(w643) -> ("Parameter"=w637:string, "DLL Interface"=w638:T6)
              n257 = Unbundle By Name(w633) -> ("Description"=w632:string)
              n258 = case shown="1" w638 {
                tunnel: [w652 w653 w654 w655 w656 w657 w658] -> w636
                tunnel: w637 -> [w652 w653 w654 w655 w656 w657 _]
                tunnel: w632 -> [_ _ _ _ _ _ w658]
                frame 0, Default {
                }
                frame 1 {
                }
                frame 2 {
                }
                frame 3 {
                }
                frame 4 {
                }
                frame 5 {
                }
                frame 6 {
                }
              }
              n259 = Not Equal?(x=w636, y="") -> (x != y?=w639:bool)
              n260 = case shown="True" w639 {
                tunnel: [-1 w665] -> w650
                tunnel: w645 -> [_ w664]
                tunnel: [errorcluster {"status"=TRUE, "code"=100, "source"="ConnectUSB: \nNo Serial Number given."} ("error in") w663] -> w641
                tunnel: w642 -> [_ w663]
                tunnel: w636 -> [_ w662]
                tunnel: w631 -> [_ w661]
                frame False {
                }
                frame True {
                  n261 = dll-call lib="T:/Entwicklung/HostSoftware/LabVIEW/GCSDrivers/source/GCS2LabVIEW/Low Level/GCSTranslator.dll" fn="ConnectUSB"(path in=w661, "ID"=w664, "szDescription"=w662) -> ("return type"=w665:i32)  [unwired: 4 in, 2 out]
                }
              }
            }
            frame "OpenRS232DaisyChain" {
              w679 = i16 0 ("width (-)")
              w691 = 12700 ("dimension size")
              # "*IDN?\nof\nconn.\ndevices"
              # "Nr. of\ndevices"
              # "OpenRS232DaisyChain"
              n262 = Decrement(x=w701) -> (x-1=w667:i32)
              n263 = global read "Global1.vi" "Interface configuration"() -> (w703:T3)
              n264 = global read "Global1.vi" "DLL device ID's"() -> (w698:i32[])
              n265 = Divide(x=w691, y=2) -> (x/y=w684:dbl)
              n266 = To Long Integer(number=w684) -> (32bit integer=w692:i32)
              n267 = Initialize Array(" ", w692) -> (w695:string[])
              n268 = Index Array(array=w703, index=w667) -> (element=w702:T4)
              n269 = Index Array(array=w698, index=w667) -> (element=w697:i32)
              n270 = Unbundle By Name(w702) -> ("RS232 Portnumber"=w704:i32, "RS232 Baud rate"=w680:u32)
              n271 = Array To Spreadsheet String(delimiter (Tab)=" ", array=w695, 3:"%s" ("format string")) -> (spreadsheet string=w689:string)
              n272 = Increment(x=w704) -> (x+1=w683:i32)
              n273 = global read "Global1.vi" "DLL Interface\nConfiguration"() -> (w672:T7)
              n274 = dll-call lib="T:/Entwicklung/HostSoftware/LabVIEW/GCSDrivers/source/GCS2LabVIEW/Low Level/GCSTranslator.dll" fn="OpenRS232DaisyChain"(path in=w666, "ID"=w697, "iPortNumber"=w683, "iBaudRate"=w680, "szBuffer"=w689, "maxlen"=w691) -> ("return type"=w677:i32, "pNrDev"=w676:i32, "szBuffer"=w675:string)  [unwired: 6 in, 3 out]
              n275 = Number To Decimal String(number=w683, width (-)=w679) -> (decimal integer string=w682:string)
              n276 = Number To Decimal String(number=w680, width (-)=w679) -> (decimal integer string=w678:string)
              n277 = call "Get lines from string.vi"("Input string"=w675) -> ("Strings"=w674:string[])  [unwired: 2 in, 16 out]
              n278 = global read "Global DaisyChain.vi" "DaisyChain configuration"() -> (w668:T9)
              n279 = Concatenate Strings("COM" ("string"), w682, "::" ("string"), w678) -> (w670:string)
              n280 = Index Array(array=w672, index=w667) -> (element=w673:T8)
              n281 = Bundle By Name(cluster=w673, "Parameter"=w670) -> (w671:T8)
              n282 = Replace Array Subset(array=w672, new element=w671, index=w667) -> (w669:T7)
              n283 = Index Array(array=w668, index=w667) -> (element=w688:T10)
              n284 = Bundle By Name(cluster=w688, "Port ID"=w677, "No. of devices"=w676, "Devices"=w674) -> (w686:T10)
              n285 = global write "Global1.vi" "DLL Interface\nConfiguration"(w669) -> ()
              n286 = Replace Array Subset(array=w668, new element=w686, index=w667) -> (w687:T9)
              n287 = global write "Global DaisyChain.vi" "DaisyChain configuration"(w687) -> ()
            }
            frame "OpenTCPIPDaisyChain" {
              w724 = 12700 ("dimension size")
              # "*IDN?\nof\nconn.\ndevices"
              # "Nr. of\ndevices"
              # "OpenTCPIPDaisyChain"
              n288 = Decrement(x=w734) -> (x-1=w706:i32)
              n289 = global read "Global1.vi" "DLL device ID's"() -> (w731:i32[])
              n290 = global read "Global1.vi" "TCP/IP Configuration"() -> (w736:T11)
              n291 = Divide(x=w724, y=2) -> (x/y=w717:dbl)
              n292 = To Long Integer(number=w717) -> (32bit integer=w725:i32)
              n293 = Initialize Array(" ", w725) -> (w728:string[])
              n294 = Index Array(array=w731, index=w706) -> (element=w730:i32)
              n295 = Index Array(array=w736, index=w706) -> (element=w735:T12)
              n296 = Array To Spreadsheet String(delimiter (Tab)=" ", array=w728, 3:"%s" ("format string")) -> (spreadsheet string=w722:string)
              n297 = Unbundle By Name(w735) -> ("Host address/name"=w711:string, "Port"=w712:i32)
              n298 = dll-call lib="T:/Entwicklung/HostSoftware/LabVIEW/GCSDrivers/source/GCS2LabVIEW/Low Level/GCSTranslator.dll" fn="OpenTCPIPDaisyChain"(path in=w705, "ID"=w730, "szHostname"=w711, "port"=w712, "szDeviceIDNs"=w722, "iBufferSize"=w724) -> ("return type"=w716:i32, "pNumberOfConnectedDaisyChainDevices"=w715:i32, "szDeviceIDNs"=w714:string)  [unwired: 5 in, 4 out]
              n299 = call "Get lines from string.vi"("Input string"=w714) -> ("Strings"=w713:string[])  [unwired: 2 in, 16 out]
              n300 = global read "Global DaisyChain.vi" "DaisyChain configuration"() -> (w720:T9)
              n301 = global read "Global1.vi" "DLL Interface\nConfiguration"() -> (w709:T7)
              n302 = Index Array(array=w720, index=w706) -> (element=w721:T10)
              n303 = Bundle By Name(cluster=w721, "Port ID"=w716, "No. of devices"=w715, "Devices"=w713) -> (w718:T10)
              n304 = Index Array(array=w709, index=w706) -> (element=w710:T8)
              n305 = Bundle By Name(cluster=w710, "Parameter"=w711) -> (w708:T8)
              n306 = Replace Array Subset(array=w709, new element=w708, index=w706) -> (w707:T7)
              n307 = Replace Array Subset(array=w720, new element=w718, index=w706) -> (w719:T9)
              n308 = global write "Global1.vi" "DLL Interface\nConfiguration"(w707) -> ()
              n309 = global write "Global DaisyChain.vi" "DaisyChain configuration"(w719) -> ()
            }
            frame "OpenUSBDaisyChain" {
              w747 = 12700 ("dimension size")
              # "*IDN?\nof\nconn.\ndevices"
              # "Nr. of\ndevices"
              # "OpenUSBDaisyChain"
              n310 = Decrement(x=w763) -> (x-1=w738:i32)
              n311 = global read "Global1.vi" "DLL Interface\nConfiguration"() -> (w743:T7)
              n312 = global read "Global1.vi" "DLL device ID's"() -> (w761:i32[])
              n313 = Index Array(array=w761, index=w738) -> (element=w760:i32)
              n314 = Divide(x=w747, y=2) -> (x/y=w752:dbl)
              n315 = To Long Integer(number=w752) -> (32bit integer=w755:i32)
              n316 = Index Array(array=w743, index=w738) -> (element=w742:T8)
              n317 = Initialize Array(" ", w755) -> (w758:string[])
              n318 = Unbundle By Name(w742) -> ("Parameter"=w741:string)
              n319 = Array To Spreadsheet String(delimiter (Tab)=" ", array=w758, 3:"%s" ("format string")) -> (spreadsheet string=w749:string)
              n320 = dll-call lib="T:/Entwicklung/HostSoftware/LabVIEW/GCSDrivers/source/GCS2LabVIEW/Low Level/GCSTranslator.dll" fn="OpenUSBDaisyChain"(path in=w737, "ID"=w760, "SN"=w741, "szBuffer"=w749, "maxlen"=w747) -> ("return type"=w751:i32, "pNrDev"=w748:i32, "szBuffer"=w746:string)  [unwired: 4 in, 4 out]
              n321 = call "Get lines from string.vi"("Input string"=w746) -> ("Strings"=w750:string[])  [unwired: 2 in, 16 out]
              n322 = global read "Global DaisyChain.vi" "DaisyChain configuration"() -> (w739:T9)
              n323 = Index Array(array=w739, index=w738) -> (element=w744:T10)
              n324 = Bundle By Name(cluster=w744, "Port ID"=w751, "No. of devices"=w748, "Devices"=w750) -> (w753:T10)
              n325 = Replace Array Subset(array=w739, new element=w753, index=w738) -> (w740:T9)
              n326 = global write "Global DaisyChain.vi" "DaisyChain configuration"(w740) -> ()
            }
            frame "ListUSB" {
              w765 = 10240 ("dimension size")
              # "*IDN?\nof\nconn.\ndevices"
              # "List USB devices"
              n327 = Decrement(x=w779) -> (x-1=w770:i32)
              n328 = global read "Global1.vi" "DLL device ID's"() -> (w776:i32[])
              n329 = Initialize Array(" ", w765) -> (w773:string[])
              n330 = Index Array(array=w776, index=w770) -> (element=w775:i32)
              n331 = Array To Spreadsheet String(delimiter (Tab)=" ", array=w773, 3:"%s" ("format string")) -> (spreadsheet string=w768:string)
              n332 = dll-call lib="T:/Entwicklung/HostSoftware/LabVIEW/GCSDrivers/source/GCS2LabVIEW/Low Level/GCSTranslator.dll" fn="ListUSB"(path in=w764, "ID"=w775, "szDescriptionList"=w768, "maxlen"=w765) -> ("return type"=w769:i32, "szDescriptionList"=w767:string)  [unwired: 4 in, 2 out]
            }
            frame "ConnectNIgpib" {
              # "Connect GPIB"
              n333 = global read "Global1.vi" "DLL device ID's"() -> (w781:i32[])
              n334 = global read "Global1.vi" "Interface configuration"() -> (w793:T3)
              n335 = Decrement(x=w791) -> (x-1=w783:i32)
              n336 = Index Array(array=w781, index=w783) -> (element=w782:i32)
              n337 = Index Array(array=w793, index=w783) -> (element=w792:T4)
              n338 = Unbundle By Name(w792) -> ("GPIB Bus"=w784:i32, "GPIB Address"=w785:i32)
              n339 = dll-call lib="T:/Entwicklung/HostSoftware/LabVIEW/GCSDrivers/source/GCS2LabVIEW/Low Level/GCSTranslator.dll" fn="ConnectNIgpib"(path in=w780, "ID"=w782, "nBoard"=w784, "nDevAddr"=w785) -> ("return type"=w790:i32)  [unwired: 5 in, 2 out]
            }
            frame "ConnectPciBoard" {
              # "Connect"
              n340 = Decrement(x=w807) -> (x-1=w795:i32)
              n341 = global read "Global1.vi" "DLL Interface\nConfiguration"() -> (w809:T7)
              n342 = global read "Global1.vi" "DLL device ID's"() -> (w798:i32[])
              n343 = Index Array(array=w798, index=w795) -> (element=w796:i32)
              n344 = Index Array(array=w809, index=w795) -> (element=w808:T8)
              n345 = Unbundle By Name(w808) -> ("Parameter"=w801:string)
              n346 = Fract/Exp String To Number(use system decimal point (T)=FALSE, string=w801) -> (number=w802:dbl)  [unwired: 3 out]
              n347 = To Long Integer(number=w802) -> (32bit integer=w797:i32)
              n348 = dll-call lib="T:/Entwicklung/HostSoftware/LabVIEW/GCSDrivers/source/GCS2LabVIEW/Low Level/GCSTranslator.dll" fn="ConnectPciBoard"(path in=w794, "ID"=w796, "iBoardNumber"=w797) -> ("return type"=w806:i32)  [unwired: 4 in, 2 out]
            }
            frame "E761_ConnectPciBoard" {
              # "E761 Connect"
              n349 = Decrement(x=w821) -> (x-1=w812:i32)
              n350 = global read "Global1.vi" "DLL Interface\nConfiguration"() -> (w823:T7)
              n351 = Index Array(array=w823, index=w812) -> (element=w822:T8)
              n352 = Unbundle By Name(w822) -> ("Parameter"=w815:string)
              n353 = Fract/Exp String To Number(use system decimal point (T)=FALSE, string=w815) -> (number=w816:dbl)  [unwired: 3 out]
              n354 = To Long Integer(number=w816) -> (32bit integer=w811:i32)
              n355 = dll-call lib="T:/Entwicklung/HostSoftware/LabVIEW/GCSDrivers/source/GCS2LabVIEW/Low Level/GCSTranslator.dll" fn="E7XX_ConnectPciBoard"(path in=w810, "IBoardNumber"=w811) -> ("return type"=w820:i32)  [unwired: 3 in, 2 out]
            }
            frame "ConnectTCPIP" {
              # "Connect TCP-IP"
              n356 = Decrement(x=w835) -> (x-1=w829:i32)
              n357 = global read "Global1.vi" "TCP/IP Configuration"() -> (w837:T11)
              n358 = global read "Global1.vi" "DLL device ID's"() -> (w830:i32[])
              n359 = Index Array(array=w837, index=w829) -> (element=w836:T12)
              n360 = Index Array(array=w830, index=w829) -> (element=w827:i32)
              n361 = Unbundle By Name(w836) -> ("Host address/name"=w826:string, "Port"=w825:i32)
              n362 = dll-call lib="T:/Entwicklung/HostSoftware/LabVIEW/GCSDrivers/source/GCS2LabVIEW/Low Level/GCSTranslator.dll" fn="ConnectTCPIP"(path in=w824, "ID"=w827, "szHostname"=w826, "port"=w825) -> ("return type"=w828:i32)  [unwired: 4 in, 3 out]
            }
            frame "GetError" {
              # "Get error"
              n363 = Decrement(x=w846) -> (x-1=w849:i32)
              n364 = global read "Global1.vi" "DLL device ID's"() -> (w848:i32[])
              n365 = Index Array(array=w848, index=w849) -> (element=w847:i32)
              n366 = dll-call lib="T:/Entwicklung/HostSoftware/LabVIEW/GCSDrivers/source/GCS2LabVIEW/Low Level/GCSTranslator.dll" fn="GetError"(path in=w838, "ID"=w847) -> ("return type"=w839:i32)  [unwired: 3 in, 2 out]
              n367 = Not Equal To 0?(x=w839) -> (x != 0?=w842:bool)
              n368 = case shown="True" w842 {
                tunnel: w841 -> [w850 w854]
                tunnel: [w850 w855] -> w840
                tunnel: w839 -> [_ w852]
                frame False {
                }
                frame True {
                  n369 = Bundle By Name(cluster=w854, "status"=TRUE, "code"=w852, "source"="GCSTranslator DLL Functions.vi: \nDLL reports error.") -> (w855:errorcluster)
                }
              }
            }
            frame "GcsCommandset" {
              # "Send string"
              n370 = Decrement(x=w861) -> (x-1=w864:i32)
              n371 = global read "Global1.vi" "DLL device ID's"() -> (w863:i32[])
              n372 = Index Array(array=w863, index=w864) -> (element=w862:i32)
              n373 = dll-call lib="T:/Entwicklung/HostSoftware/LabVIEW/GCSDrivers/source/GCS2LabVIEW/Low Level/GCSTranslator.dll" fn="GcsCommandset"(path in=w856, "ID"=w862, "szCommand"=w859) -> ("return type"=w865:i32)  [unwired: 4 in, 2 out]
            }
            frame "GCSGetAnswerSize" {
              # "Get number of bytes to read"
              n374 = Decrement(x=w871) -> (x-1=w874:i32)
              n375 = global read "Global1.vi" "DLL device ID's"() -> (w873:i32[])
              n376 = Index Array(array=w873, index=w874) -> (element=w872:i32)
              n377 = dll-call lib="T:/Entwicklung/HostSoftware/LabVIEW/GCSDrivers/source/GCS2LabVIEW/Low Level/GCSTranslator.dll" fn="GcsGetAnswerSize"(path in=w867, "ID"=w872, "iAnswerSize"=0) -> ("return type"=w875:i32, "iAnswerSize"=w869:i32)  [unwired: 3 in, 2 out]
            }
            frame "GcsGetAnswer" {
              # "Get answer string"
              n378 = Decrement(x=w884) -> (x-1=w887:i32)
              n379 = global read "Global1.vi" "DLL device ID's"() -> (w886:i32[])
              n380 = Index Array(array=w886, index=w887) -> (element=w885:i32)
              n381 = dll-call lib="T:/Entwicklung/HostSoftware/LabVIEW/GCSDrivers/source/GCS2LabVIEW/Low Level/GCSTranslator.dll" fn="GcsGetAnswer"(path in=w878, "ID"=w885, "szAnswer"=w882, "iAnswerSize"=w879) -> ("return type"=w888:i32, "szAnswer"=w881:string)  [unwired: 4 in, 2 out]
            }
          }
        }
        frame condition #1 {
        }
        frame condition #2 {
        }
      }
    }
    frame Error {
    }
  }
  "error out" <- w12
  "DLL I32 Return value" <- w11
  "Boolean output" <- w10
  "Numerical output" <- w8
  "String output" <- w6
